vi "Host_test_webdav.vi"() -> ()   [LabVIEW 2025]
panel:
  out "dowloads":string[](array[string])
  out "error out":errorcluster
  in  "local file path":path
  in  "password":string
  in  "user":string
  in  "IP myRIO":string="172.22.11.2"
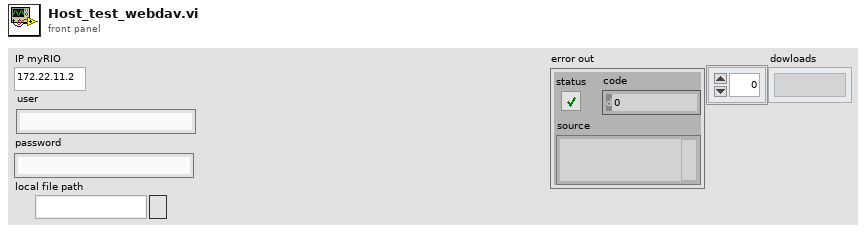
[diagram p1: front panel]
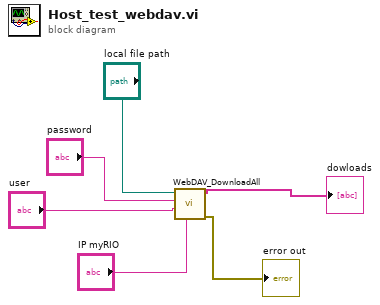
[diagram p0: block diagram]
diagram:
  n1 = call "WebDAV_DownloadAll.vi"("IP myRIO"="IP myRIO", "user"="user", "password"="password", "local file path"="local file path") -> ("error out"=→"error out":errorcluster, "dowloads"=→"dowloads":string[])  [unwired: 6 in]
